vi "Add Meas Plugin Indicators.vi"(11 "error in (no error)":errorcluster) -> (15 "error out":errorcluster)   [LabVIEW 2021, in "Migrator.lvlib"]
uses:
  Migrator.lvlib
  Migrator Reusables/Migrator Reusables.lvlib
  Path Functions/Path Functions.lvlib
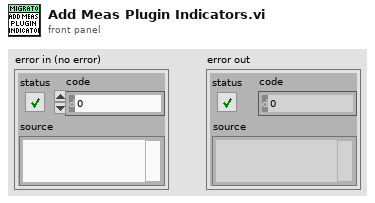
[diagram p1: front panel]
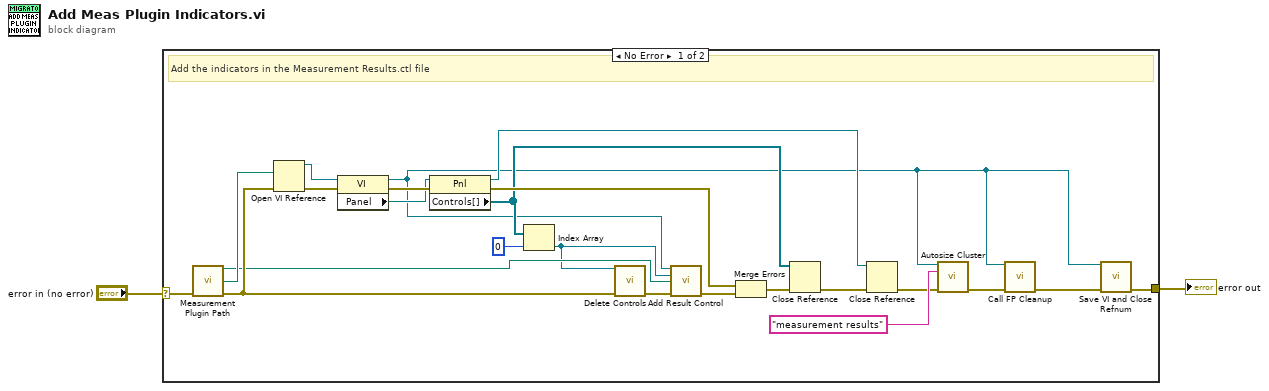
[diagram p0: block diagram]
diagram:
  n1 = case shown="No Error" "error in (no error)" {
    selector: "error in (no error)" -> [w9 w26]
    tunnel: [w19 w26] -> w2
    frame No Error {
      # "Add the indicators in the Measurement Results.ctl file"
      n2 = call "Measurement Plugin Path.vi"("error in (no error)"=w9) -> ("New Code Module"=w5:path, "Result Control"=w10:path, "error out"=w8:errorcluster)  [unwired: 2 in, 10 out]
      n3 = Open VI Reference(vi path=w10, error in (no error)=w8) -> (vi reference=w11:refnum<vi>, error out=w22:errorcluster)  [unwired: 4 in]
      n4 = property class="VI"(reference=w11, error in=w22) -> (reference out=w3:refnum<vi>, error out=w25:errorcluster, "Panel"=w23:refnum<vi>)
      n5 = property class="Pnl"(reference=w23, error in=w25) -> (reference out=w16:refnum<vi>, error out=w15:errorcluster, "Controls[]"=w14:refnum<vi>[])
      n6 = Index Array(array=w14, index=0) -> (element=w4:refnum<vi>)
      n7 = call "Delete Controls.vi"("Control in"=w4, "error in (no error)"=w8) -> ("error out"=w7:errorcluster)  [unwired: 13 in]
      n8 = call "Add Result Control.vi"("VI Reference"=w3, "Result Cluster"=w4, "New Code Module"=w5, "error in (no error)"=w7) -> ("error out"=w6:errorcluster)  [unwired: 11 in]
      n9 = Merge Errors(w15, w6) -> (w13:errorcluster)
      n10 = Close Reference(reference=w14, error in (no error)=w13) -> (error out=w12:errorcluster)
      n11 = Close Reference(reference=w16, error in (no error)=w12) -> (error out=w20:errorcluster)
      n12 = call "Autosize Cluster.vi"("VI Refnum"=w3, "name"="measurement results" ("name/order"), "error in (no error)"=w20) -> ("error out"=w18:errorcluster)  [unwired: 12 in]
      n13 = call "Call FP Cleanup.vi"("VI"=w3, "error in (no error)"=w18) -> ("error out"=w17:errorcluster)  [unwired: 13 in]
      n14 = call "Save VI and Close Refnum.vi"("VI Refnum"=w3, "error in"=w17) -> ("error out"=w19:errorcluster)  [unwired: 13 in]
    }
    frame Error {
    }
  }
  "error out" <- w2
